vi "Label of File Name Array in Hash List--constant.vi"() -> (3 "Label of File Name Array in Hash List":string)   [LabVIEW 2026]
doc: "Label of file name array in hash list constant."
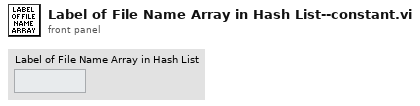
[diagram p1: front panel]
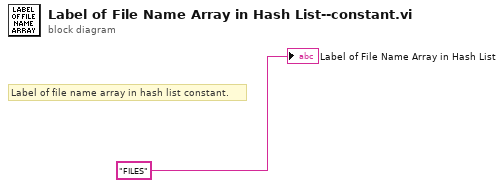
[diagram p0: block diagram]
diagram:
  # "Label of file name array in hash list constant."
  "Label of File Name Array in Hash List" <- "FILES" ("Label of File Name Array in Hash List")
